vi "Battery_Test_System_Main.vi"() -> ()   [LabVIEW 2019]
doc: "Battery Test System - SIMULATION MODE. One While Loop: Event Structure (UI commands, timeout = UI Update Interval) -> state Case Structure (INIT, IDLE/STOPPED/FAULT, CHARGING/DISCHARGING completion, Default safe fallback) -> Sim_Update_Model (simulated sensor source and output interlock) -> Sim_Check_Safety (latched faults) -> bounded log -> XY graphs and indicators. dt is measured with Tick Count and clamped to Max dt. No physical I/O anywhere. All limits are DEMONSTRATION values only."
uses:
  Sim_Settings.ctl
  Test_State_Enum2.ctl
  Sim_State_Enum.ctl
panel:
  out "Status Message":string
  out "Fault Message":string
  out "Fault":bool
  out "Sim DC Load Output":bool
  out "Sim Power Supply Output":bool
  out "Cycle Count":u32
  out "Elapsed Time (s)":dbl
  out "Temperature (degC)":dbl
  out "DC Current (A)":dbl
  out "DC Voltage (V)":dbl
  out "SOC (%)":dbl
  out "Temperature Graph":T1(graph)
  out "DC Current Graph":cluster{"Time (s)":dbl[], "Current (A)":dbl[]}(graph)
  out "DC Voltage Graph":cluster{"Time (s)":dbl[], "Voltage (V)":dbl[]}(graph)
  out "Current State":T2
  in  "Close":bool
  in  "Reset Fault":bool
  in  "Save":bool
  in  "Stop":bool
  in  "Discharge Settings":T3={"Voltage (V)"=11.0, "Current (A)"=5.0, "C-Rate (1/h)"=1.0, "Duration (min)"=10.0}
  in  "Charge Settings":T3={"Voltage (V)"=14.0, "Current (A)"=5.0, "C-Rate (1/h)"=1.0, "Duration (min)"=10.0}
  in  "Start":bool
  in  "Operation Mode":T4
  in  "Simulation Settings (DEMO ONLY)":T5={"UI Update Interval (ms)"=200, "Max dt (s)"=1.0, "Initial SOC (%)"=50.0, "Rest Voltage (V)"=12.0, "Ambient Temperature (degC)"=25.0, "Voltage Time Constant (s)"=5.0, "Current Time Constant (s)"=1.0, "Thermal Time Constant (s)"=120.0, "Heating Coefficient (degC/s per A^2)"=0.002, "SOC Speed Factor"=1.0, "Charge Complete SOC (%)"=100.0, "Discharge Complete SOC (%)"=0.0, "Max Voltage Limit (V)"=15.0, "Max Current Limit (A)"=10.0, "Max Temperature Limit (degC)"=45.0, "Max C-Rate (1/h)"=5.0, "Max Duration (min)"=600.0, "History Length (samples)"=3000, "Inject E-Stop"=FALSE, "Inject Overvoltage"=FALSE, "Inject Overcurrent"=FALSE, "Inject Overtemperature"=FALSE}
  out "DC Load Connected?":bool
  out "Power Supply Connected?":bool
  out "DAQ CONNECTED?":bool
  out "SIMULATION MODE":string
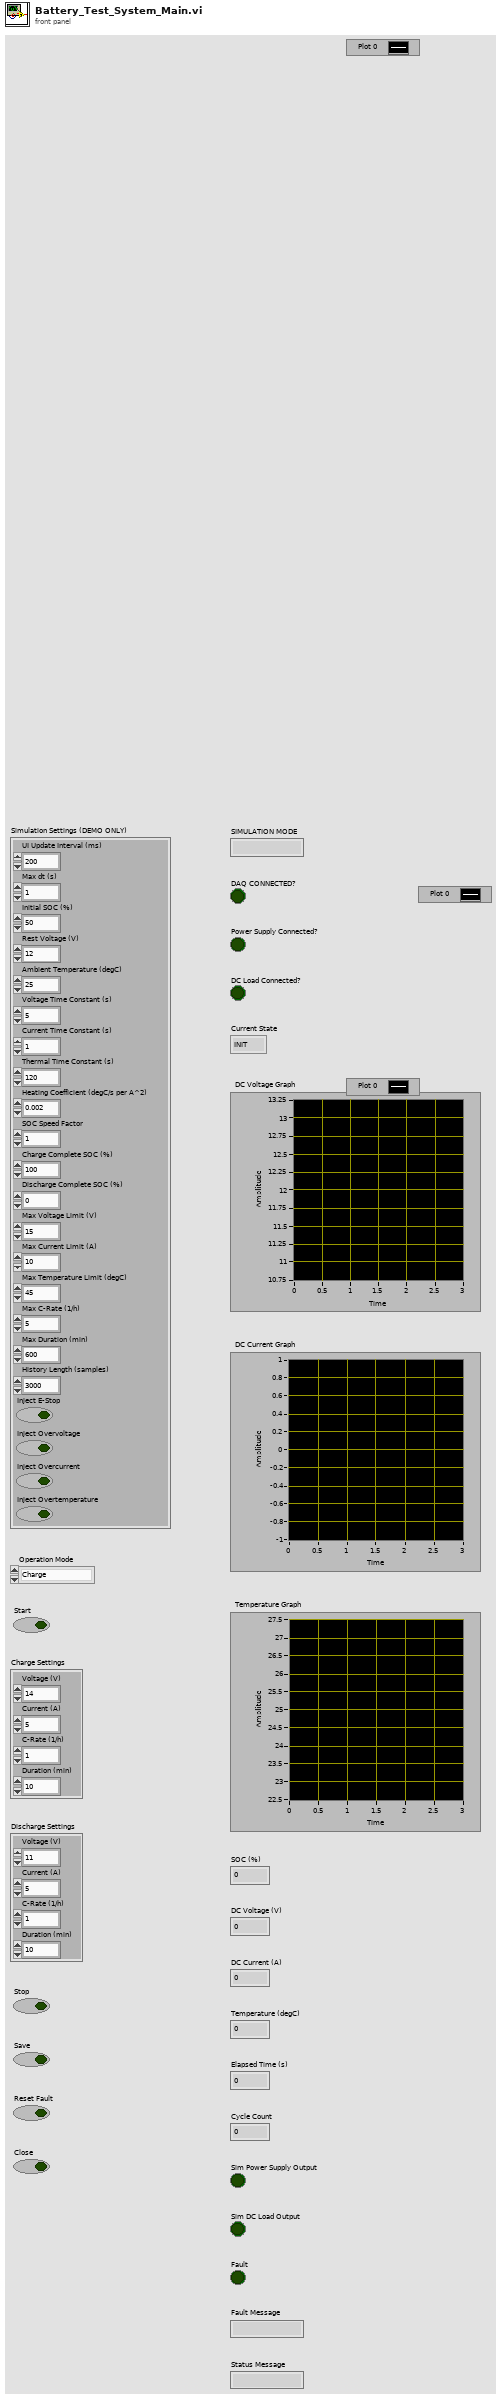
[diagram p1: front panel]
types:
  T1 = cluster{"Time (s)":dbl[], "Temperature (degC)":dbl[]}
  T2 = typedef "Sim_State_Enum.ctl" = enum16{"INIT", "IDLE", "CHARGING", "DISCHARGING", "STOPPED", "FAULT"}
  T3 = cluster{"Voltage (V)":dbl, "Current (A)":dbl, "C-Rate (1/h)":dbl, "Duration (min)":dbl}
  T4 = typedef "Test_State_Enum2.ctl" = enum16{"Charge", "Discharge"}
  T5 = typedef "Sim_Settings.ctl" = cluster{"UI Update Interval (ms)":i32, "Max dt (s)":dbl, "Initial SOC (%)":dbl, "Rest Voltage (V)":dbl, "Ambient Temperature (degC)":dbl, "Voltage Time Constant (s)":dbl, "Current Time Constant (s)":dbl, "Thermal Time Constant (s)":dbl, "Heating Coefficient (degC/s per A^2)":dbl, "SOC Speed Factor":dbl, "Charge Complete SOC (%)":dbl, "Discharge Complete SOC (%)":dbl, "Max Voltage Limit (V)":dbl, "Max Current Limit (A)":dbl, "Max Temperature Limit (degC)":dbl, "Max C-Rate (1/h)":dbl, "Max Duration (min)":dbl, "History Length (samples)":i32, "Inject E-Stop":bool, "Inject Overvoltage":bool, "Inject Overcurrent":bool, "Inject Overtemperature":bool}
  T6 = cluster{"Timestamp":string, "State":enum16{"INIT", "IDLE", "CHARGING", "DISCHARGING", "STOPPED", "FAULT"}, "Data":cluster{"SOC (%)":dbl, "Voltage (V)":dbl, "Current (A)":dbl, "Temperature (degC)":dbl, "Run Time (s)":dbl, "Elapsed (s)":dbl, "Cycle Count":u32, "Active Mode":enum16{"Charge", "Discharge"}, "Setpoint Voltage (V)":dbl, "Setpoint Current (A)":dbl, "Setpoint C-Rate (1/h)":dbl, "Setpoint Duration (min)":dbl, "Sim PS Enable":bool, "Sim Load Enable":bool, "Charge Half Done":bool, "Discharge Half Done":bool, "Fault":bool, "Fault Code":i32, "Fault Message":string, "Fault Time":string, "Status Message":string}}[]
  T7 = cluster{"SOC (%)":dbl, "Voltage (V)":dbl, "Current (A)":dbl, "Temperature (degC)":dbl, "Run Time (s)":dbl, "Elapsed (s)":dbl, "Cycle Count":u32, "Active Mode":enum16{"Charge", "Discharge"}, "Setpoint Voltage (V)":dbl, "Setpoint Current (A)":dbl, "Setpoint C-Rate (1/h)":dbl, "Setpoint Duration (min)":dbl, "Sim PS Enable":bool, "Sim Load Enable":bool, "Charge Half Done":bool, "Discharge Half Done":bool, "Fault":bool, "Fault Code":i32, "Fault Message":string, "Fault Time":string, "Status Message":string}
  T8 = enum16{"INIT", "IDLE", "CHARGING", "DISCHARGING", "STOPPED", "FAULT"}
  T9 = cluster{"Timestamp":string, "State":enum16{"INIT", "IDLE", "CHARGING", "DISCHARGING", "STOPPED", "FAULT"}, "Data":cluster{"SOC (%)":dbl, "Voltage (V)":dbl, "Current (A)":dbl, "Temperature (degC)":dbl, "Run Time (s)":dbl, "Elapsed (s)":dbl, "Cycle Count":u32, "Active Mode":enum16{"Charge", "Discharge"}, "Setpoint Voltage (V)":dbl, "Setpoint Current (A)":dbl, "Setpoint C-Rate (1/h)":dbl, "Setpoint Duration (min)":dbl, "Sim PS Enable":bool, "Sim Load Enable":bool, "Charge Half Done":bool, "Discharge Half Done":bool, "Fault":bool, "Fault Code":i32, "Fault Message":string, "Fault Time":string, "Status Message":string}}
  T10 = typedef "Sim_Data.ctl" = cluster{"SOC (%)":dbl, "Voltage (V)":dbl, "Current (A)":dbl, "Temperature (degC)":dbl, "Run Time (s)":dbl, "Elapsed (s)":dbl, "Cycle Count":u32, "Active Mode":T4, "Setpoint Voltage (V)":dbl, "Setpoint Current (A)":dbl, "Setpoint C-Rate (1/h)":dbl, "Setpoint Duration (min)":dbl, "Sim PS Enable":bool, "Sim Load Enable":bool, "Charge Half Done":bool, "Discharge Half Done":bool, "Fault":bool, "Fault Code":i32, "Fault Message":string, "Fault Time":string, "Status Message":string}
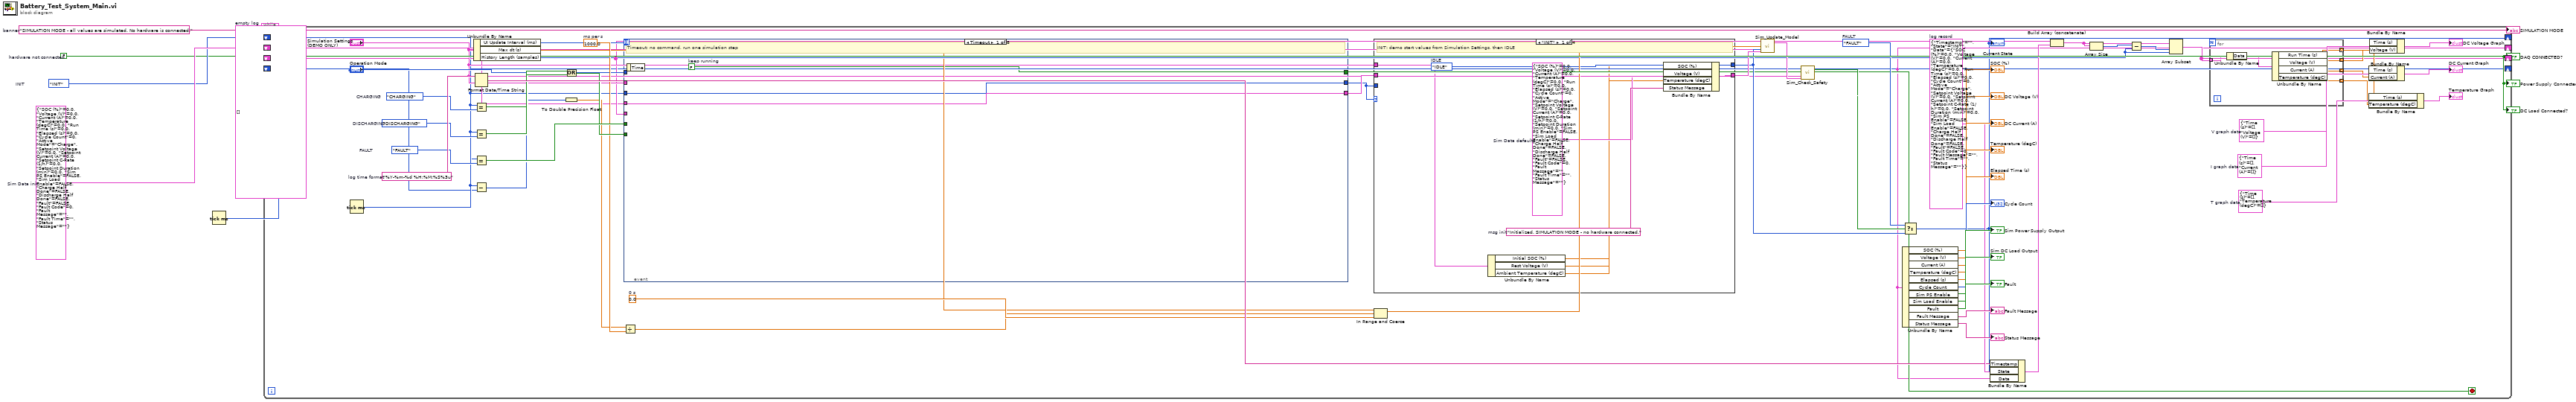
[diagram p0: block diagram]
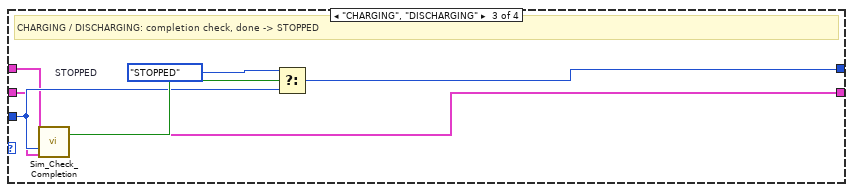
[diagram p3: hidden frame]
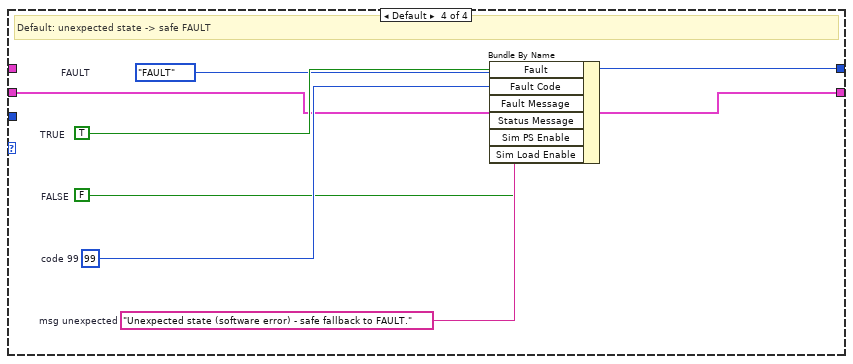
[diagram p4: hidden frame]
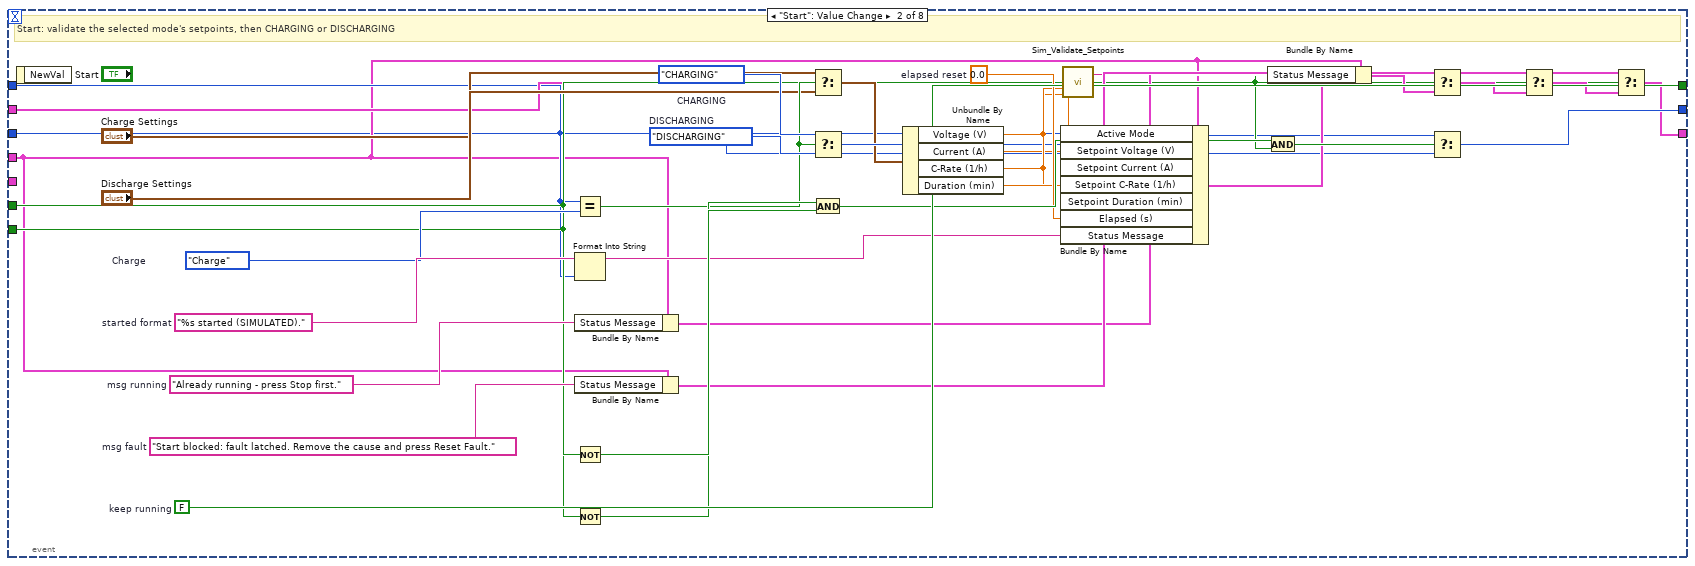
[diagram p5: hidden frame]
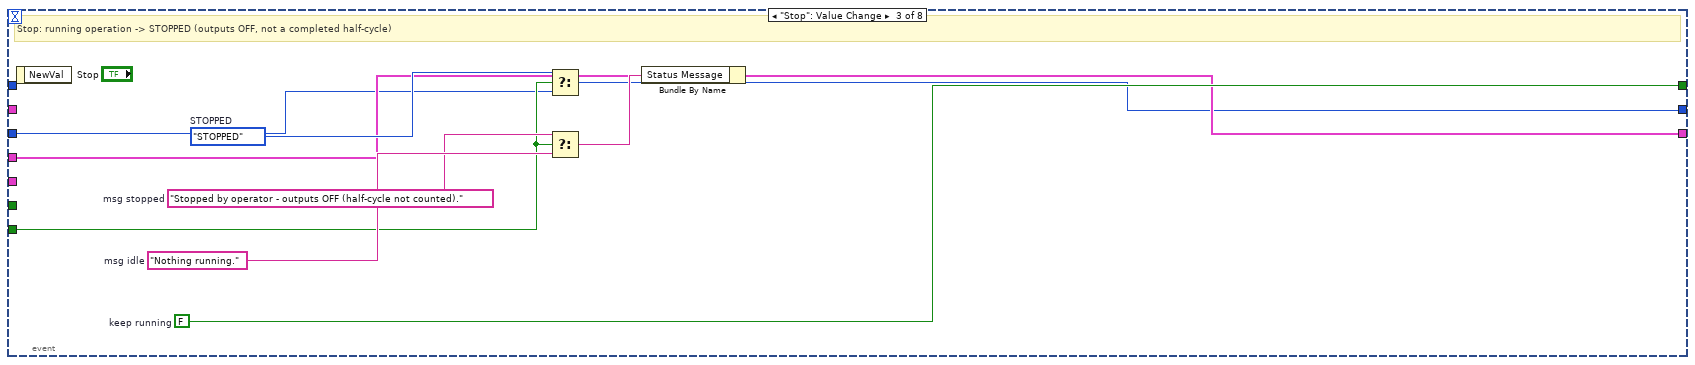
[diagram p6: hidden frame]
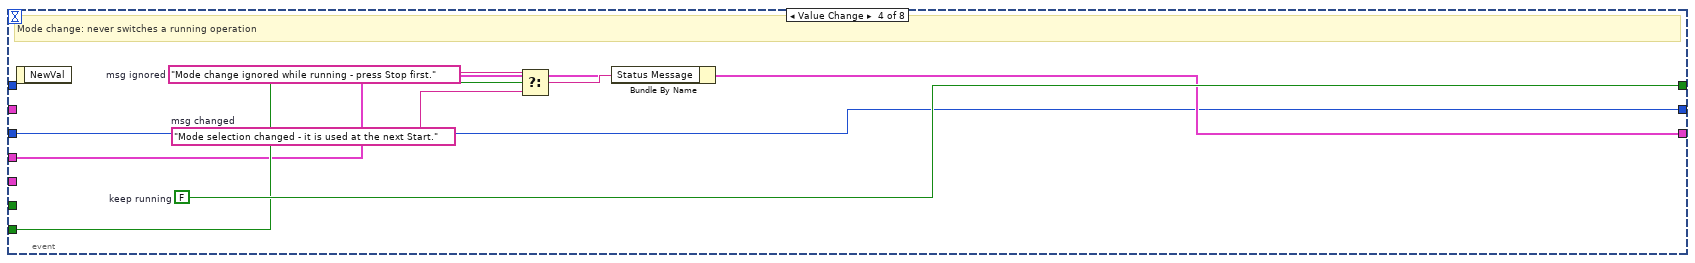
[diagram p7: hidden frame]
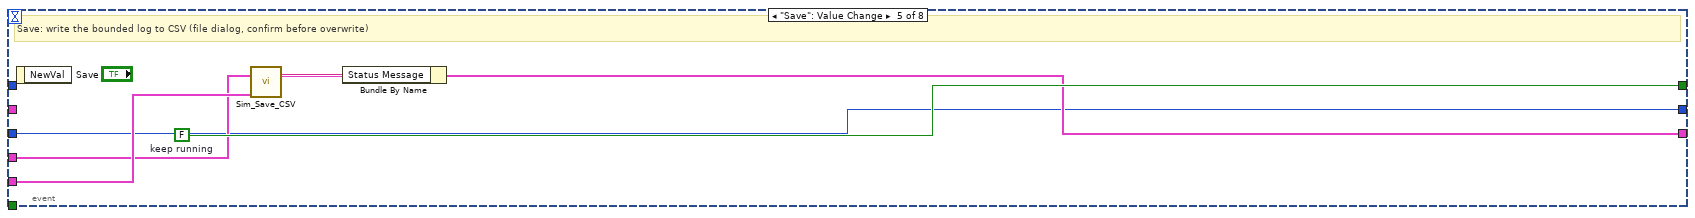
[diagram p8: hidden frame]
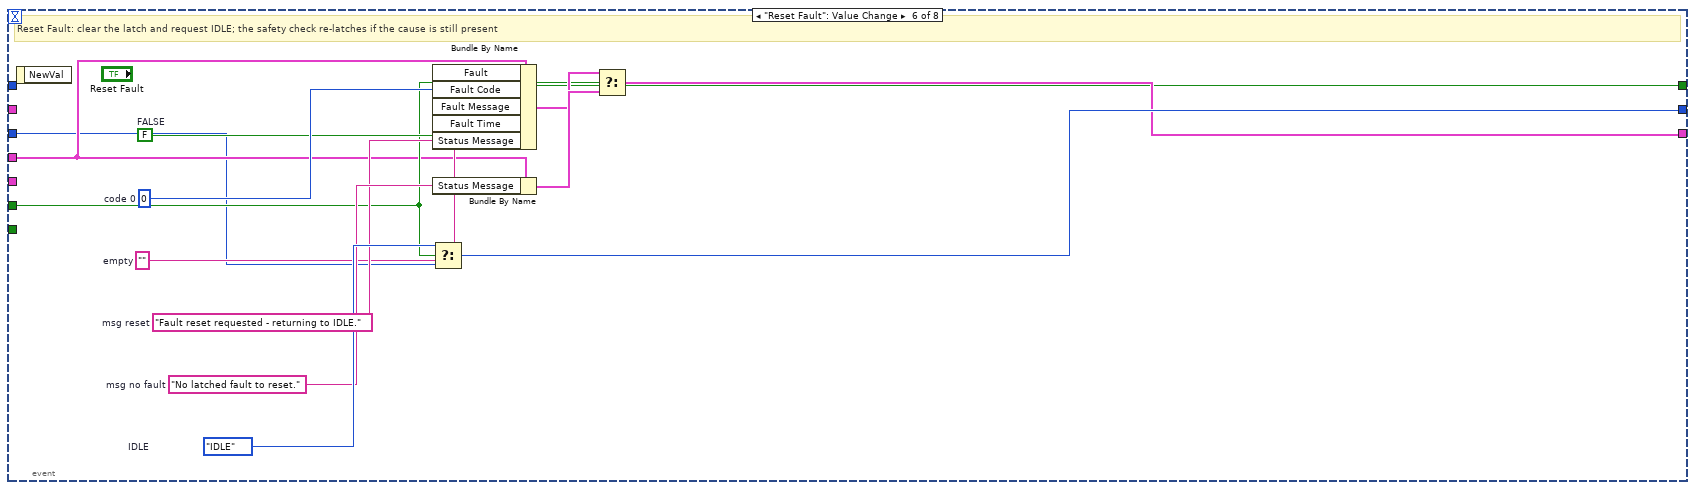
[diagram p9: hidden frame]
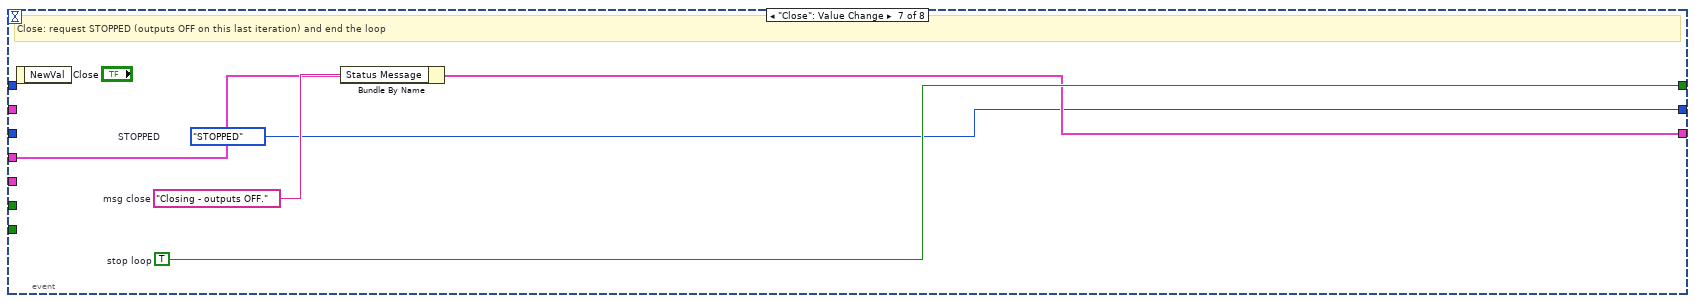
[diagram p10: hidden frame]
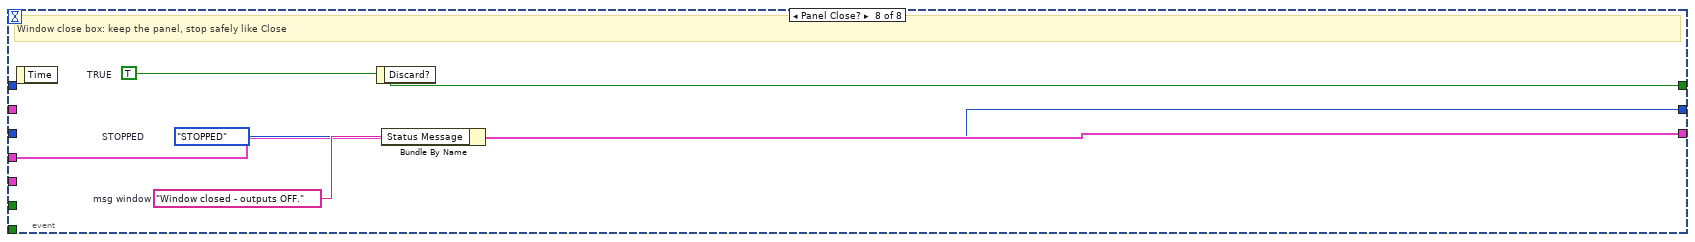
[diagram p11: hidden frame]
diagram:
  w6 = T6 []  # empty log
  w4 = T7 {"SOC (%)"=0.0, "Voltage (V)"=0.0, "Current (A)"=0.0, "Temperature (degC)"=0.0, "Run Time (s)"=0.0, "Elapsed (s)"=0.0, "Cycle Count"=0, "Active Mode"=enum."Charge", "Setpoint Voltage (V)"=0.0, "Setpoint Current (A)"=0.0, "Setpoint C-Rate (1/h)"=0.0, "Setpoint Duration (min)"=0.0, "Sim PS Enable"=FALSE, "Sim Load Enable"=FALSE, "Charge Half Done"=FALSE, "Discharge Half Done"=FALSE, "Fault"=FALSE, "Fault Code"=0, "Fault Message"="", "Fault Time"="", "Status Message"=""}  # Sim Data init
  w3 = T8."INIT"  # INIT
  w2 = FALSE  # hardware not connected
  w1 = "SIMULATION MODE - all values are simulated. No hardware is connected."  # banner
  n1 = Tick Count (ms)() -> (millisecond timer value=w5:u32)
  n2 = while {
    shift-right: [w8] -> _
    shift-left: w3 -> [w7]
    shift-right: [w10] -> _
    shift-left: w4 -> [w9]
    shift-right: [w14] -> _
    shift-left: w6 -> [w13]
    shift-right: [w12] -> _
    shift-left: w5 -> [w11]
    stop <- w35 stop-if-true
    w56 = T1 {"Time (s)"=[], "Temperature (degC)"=[]}  # T graph data
    w54 = cluster{"Time (s)":dbl[], "Current (A)":dbl[]} {"Time (s)"=[], "Current (A)"=[]}  # I graph data
    w52 = cluster{"Time (s)":dbl[], "Voltage (V)":dbl[]} {"Time (s)"=[], "Voltage (V)"=[]}  # V graph data
    w43 = T9 {"Timestamp"="", "State"=enum."INIT", "Data"={"SOC (%)"=0.0, "Voltage (V)"=0.0, "Current (A)"=0.0, "Temperature (degC)"=0.0, "Run Time (s)"=0.0, "Elapsed (s)"=0.0, "Cycle Count"=0, "Active Mode"=enum."Charge", "Setpoint Voltage (V)"=0.0, "Setpoint Current (A)"=0.0, "Setpoint C-Rate (1/h)"=0.0, "Setpoint Duration (min)"=0.0, "Sim PS Enable"=FALSE, "Sim Load Enable"=FALSE, "Charge Half Done"=FALSE, "Discharge Half Done"=FALSE, "Fault"=FALSE, "Fault Code"=0, "Fault Message"="", "Fault Time"="", "Status Message"=""}}  # log record
    w41 = "%Y-%m-%d %H:%M:%S%3u"  # log time format
    w40 = T8."FAULT"  # FAULT
    w28 = T8."FAULT"  # FAULT
    w27 = T8."DISCHARGING"  # DISCHARGING
    w26 = T8."CHARGING"  # CHARGING
    w24 = 0.0  # 0 s
    w22 = 1000.0  # ms per s
    n3 = Tick Count (ms)() -> (millisecond timer value=w12:u32)
    n4 = Unbundle By Name("Simulation Settings (DEMO ONLY)") -> ("UI Update Interval (ms)"=w17:i32, "Max dt (s)"=w18:dbl, "History Length (samples)"=w19:i32)
    n5 = Format Date/Time String(time format string (%c)=w41) -> (date/time string=w42:string)  [unwired: 1 in, 1 out]
    n6 = Equal?(x=w7, y=w26) -> (x = y?=w29:bool)
    n7 = Equal?(x=w7, y=w27) -> (x = y?=w30:bool)
    n8 = Equal?(x=w7, y=w28) -> (x = y?=w32:bool)
    n9 = Subtract(x=w12, y=w11) -> (x-y=w20:u32)
    n10 = Or(x=w29, y=w30) -> (x .or. y?=w31:bool)
    n11 = To Double Precision Float(number=w20) -> (double precision float=w21:dbl)
    n12 = event shown="[0] Timeout" {
      selector: _ -> [_ _ _ _ _ _ _ _]
      dyn-events: _ -> [_ _ _ _ _ _ _ _]
      timeout: w17 -> [_ _ _ _ _ _ _ _]
      tunnel: "Operation Mode" -> [_ w104 _ _ _ _ _ _]
      tunnel: "Simulation Settings (DEMO ONLY)" -> [_ w105 _ _ _ _ _ _]
      tunnel: [w101 w139 w149 w157 w163 w167 w181 w183] -> w35
      tunnel: w7 -> [w99 w102 w140 w150 w158 w164 _ _]
      tunnel: w9 -> [w100 w103 w141 w151 w159 w165 w177 w182]
      tunnel: w13 -> [_ _ _ _ w160 _ _ _]
      tunnel: w32 -> [_ w107 _ _ _ w166 _ _]
      tunnel: [w99 w138 w144 w150 w158 w176 w178 w184] -> w33
      tunnel: [w100 w133 w148 w156 w162 w174 w180 w186] -> w34
      tunnel: w31 -> [_ w106 w142 w152 _ _ _ _]
      event Timeout {
        w101 = FALSE  # keep running
        # "Timeout: no command, run one simulation step"
        n13 = event-data() -> ()  [unwired: 1 in, 1 out]
      }
      event "Start": Value Change {
        w139 = FALSE  # keep running
        w129 = "Start blocked: fault latched. Remove the cause and press Reset Fault."  # msg fault
        w127 = "Already running - press Stop first."  # msg running
        w124 = 0.0  # elapsed reset
        w122 = "%s started (SIMULATED)."  # started format
        w114 = T8."DISCHARGING"  # DISCHARGING
        w113 = T8."CHARGING"  # CHARGING
        w110 = enum16{"Charge", "Discharge"}."Charge"  # Charge
        # "Start: validate the selected mode's setpoints, then CHARGING or DISCHARGING"
        n14 = event-data() -> ()  [unwired: 1 in, 1 out]
        n15 = Equal?(x=w104, y=w110) -> (x = y?=w111:bool)
        n16 = Format Into String(format string=w122, w104) -> (resulting string=w123:string)  [unwired: 2 in, 1 out]
        n17 = Bundle By Name(cluster=w103, "Status Message"=w127) -> (w128:T10)
        n18 = Bundle By Name(cluster=w103, "Status Message"=w129) -> (w130:T10)
        n19 = Not(x=w107) -> (.not. x?=w135:bool)
        n20 = Not(x=w106) -> (.not. x?=w134:bool)
        n21 = Select(t="Charge Settings", s=w111, f="Discharge Settings") -> (s? t:f=w112:T3)
        n22 = Select(t=w113, s=w111, f=w114) -> (s? t:f=w115:T8)
        n23 = And(x=w134, y=w135) -> (x .and. y?=w136:bool)
        n24 = Unbundle By Name(w112) -> ("Voltage (V)"=w116:dbl, "Current (A)"=w117:dbl, "C-Rate (1/h)"=w118:dbl, "Duration (min)"=w119:dbl)
        n25 = Bundle By Name(cluster=w103, "Active Mode"=w104, "Setpoint Voltage (V)"=w116, "Setpoint Current (A)"=w117, "Setpoint C-Rate (1/h)"=w118, "Setpoint Duration (min)"=w119, "Elapsed (s)"=w124, "Status Message"=w123) -> (w125:T10)
        n26 = call "Sim_Validate_Setpoints.vi"("Settings"=w105, "Duration (min)"=w119, "C-Rate (1/h)"=w118, "Current (A)"=w117, "Voltage (V)"=w116) -> ("Message"=w121:string, "Valid?"=w120:bool)  [unwired: 9 in]
        n27 = Bundle By Name(cluster=w103, "Status Message"=w121) -> (w126:T10)
        n28 = And(x=w136, y=w120) -> (x .and. y?=w137:bool)
        n29 = Select(t=w125, s=w120, f=w126) -> (s? t:f=w131:T10)
        n30 = Select(t=w115, s=w137, f=w102) -> (s? t:f=w138:T8)
        n31 = Select(t=w130, s=w107, f=w131) -> (s? t:f=w132:T10)
        n32 = Select(t=w128, s=w106, f=w132) -> (s? t:f=w133:T10)
      }
      event "Stop": Value Change {
        w149 = FALSE  # keep running
        w146 = "Nothing running."  # msg idle
        w145 = "Stopped by operator - outputs OFF (half-cycle not counted)."  # msg stopped
        w143 = T8."STOPPED"  # STOPPED
        # "Stop: running operation -> STOPPED (outputs OFF, not a completed half-cycle)"
        n33 = event-data() -> ()  [unwired: 1 in, 1 out]
        n34 = Select(t=w143, s=w142, f=w140) -> (s? t:f=w144:T8)
        n35 = Select(t=w145, s=w142, f=w146) -> (s? t:f=w147:string)
        n36 = Bundle By Name(cluster=w141, "Status Message"=w147) -> (w148:T10)
      }
      event Value Change {
        w157 = FALSE  # keep running
        w154 = "Mode selection changed - it is used at the next Start."  # msg changed
        w153 = "Mode change ignored while running - press Stop first."  # msg ignored
        # "Mode change: never switches a running operation"
        n37 = event-data() -> ()  [unwired: 1 in, 1 out]
        n38 = Select(t=w153, s=w152, f=w154) -> (s? t:f=w155:string)
        n39 = Bundle By Name(cluster=w151, "Status Message"=w155) -> (w156:T10)
      }
      event "Save": Value Change {
        w163 = FALSE  # keep running
        # "Save: write the bounded log to CSV (file dialog, confirm before overwrite)"
        n40 = event-data() -> ()  [unwired: 1 in, 1 out]
        n41 = call "Sim_Save_CSV.vi"("Log Records"=w160) -> ("Status Message"=w161:string)  [unwired: 13 in, 1 out]
        n42 = Bundle By Name(cluster=w159, "Status Message"=w161) -> (w162:T10)
      }
      event "Reset Fault": Value Change {
        w175 = T8."IDLE"  # IDLE
        w171 = "No latched fault to reset."  # msg no fault
        w170 = "Fault reset requested - returning to IDLE."  # msg reset
        w169 = ""  # empty
        w168 = 0  # code 0
        w167 = FALSE  # FALSE
        # "Reset Fault: clear the latch and request IDLE; the safety check re-latches if the cause is still present"
        n43 = event-data() -> ()  [unwired: 1 in, 1 out]
        n44 = Bundle By Name(cluster=w165, "Fault"=w167, "Fault Code"=w168, "Fault Message"=w169, "Fault Time"=w169, "Status Message"=w170) -> (w172:T10)
        n45 = Bundle By Name(cluster=w165, "Status Message"=w171) -> (w173:T10)
        n46 = Select(t=w175, s=w166, f=w164) -> (s? t:f=w176:T8)
        n47 = Select(t=w172, s=w166, f=w173) -> (s? t:f=w174:T10)
      }
      event "Close": Value Change {
        w181 = TRUE  # stop loop
        w179 = "Closing - outputs OFF."  # msg close
        w178 = T8."STOPPED"  # STOPPED
        # "Close: request STOPPED (outputs OFF on this last iteration) and end the loop"
        n48 = event-data() -> ()  [unwired: 1 in, 1 out]
        n49 = Bundle By Name(cluster=w177, "Status Message"=w179) -> (w180:T10)
      }
      event Panel Close? {
        w185 = "Window closed - outputs OFF."  # msg window
        w184 = T8."STOPPED"  # STOPPED
        w183 = TRUE  # TRUE
        # "Window close box: keep the panel, stop safely like Close"
        n50 = event-data() -> ()  [unwired: 1 in, 1 out]
        n51 = event-data("Discard?"=w183) -> ()  [unwired: 1 in, 1 out]
        n52 = Bundle By Name(cluster=w182, "Status Message"=w185) -> (w186:T10)
      }
    }
    n53 = Divide(x=w21, y=w22) -> (x/y=w23:dbl)
    n54 = case shown="\"INIT\"" w33 {
      tunnel: "Simulation Settings (DEMO ONLY)" -> [w75 _ w86 _]
      tunnel: [w82 w84 w91 w93] -> w36
      tunnel: w34 -> [_ w83 w85 w92]
      tunnel: w33 -> [_ w84 w87 _]
      tunnel: [w81 w83 w88 w98] -> w37
      frame "INIT" {
        w82 = T8."IDLE"  # IDLE
        w80 = "Initialized. SIMULATION MODE - no hardware connected."  # msg init
        w79 = T7 {"SOC (%)"=0.0, "Voltage (V)"=0.0, "Current (A)"=0.0, "Temperature (degC)"=0.0, "Run Time (s)"=0.0, "Elapsed (s)"=0.0, "Cycle Count"=0, "Active Mode"=enum."Charge", "Setpoint Voltage (V)"=0.0, "Setpoint Current (A)"=0.0, "Setpoint C-Rate (1/h)"=0.0, "Setpoint Duration (min)"=0.0, "Sim PS Enable"=FALSE, "Sim Load Enable"=FALSE, "Charge Half Done"=FALSE, "Discharge Half Done"=FALSE, "Fault"=FALSE, "Fault Code"=0, "Fault Message"="", "Fault Time"="", "Status Message"=""}  # Sim Data defaults
        # "INIT: demo start values from Simulation Settings, then IDLE"
        n55 = Unbundle By Name(w75) -> ("Initial SOC (%)"=w76:dbl, "Rest Voltage (V)"=w77:dbl, "Ambient Temperature (degC)"=w78:dbl)
        n56 = Bundle By Name(cluster=w79, "SOC (%)"=w76, "Voltage (V)"=w77, "Temperature (degC)"=w78, "Status Message"=w80) -> (w81:T7)
      }
      frame "IDLE", "STOPPED", "FAULT" {
        # "IDLE / STOPPED / FAULT: hold; the model forces both outputs OFF"
      }
      frame "CHARGING", "DISCHARGING" {
        w90 = T8."STOPPED"  # STOPPED
        # "CHARGING / DISCHARGING: completion check, done -> STOPPED"
        n57 = call "Sim_Check_Completion.vi"("State"=w87, "Settings"=w86, "Sim Data in"=w85) -> ("Done?"=w89:bool, "Sim Data out"=w88:T10)  [unwired: 11 in]
        n58 = Select(t=w90, s=w89, f=w87) -> (s? t:f=w91:T8)
      }
      frame Default {
        w97 = "Unexpected state (software error) - safe fallback to FAULT."  # msg unexpected
        w96 = 99  # code 99
        w95 = FALSE  # FALSE
        w94 = TRUE  # TRUE
        w93 = T8."FAULT"  # FAULT
        # "Default: unexpected state -> safe FAULT"
        n59 = Bundle By Name(cluster=w92, "Fault"=w94, "Fault Code"=w96, "Fault Message"=w97, "Status Message"=w97, "Sim PS Enable"=w95, "Sim Load Enable"=w95) -> (w98:T10)
      }
    }
    n60 = In Range and Coerce(upper limit=w18, x=w23, lower limit=w24) -> (coerced(x)=w25:dbl)  [unwired: 1 out]
    n61 = call "Sim_Update_Model.vi"("dt (s)"=w25, "State"=w36, "Settings"="Simulation Settings (DEMO ONLY)", "Sim Data in"=w37) -> ("Sim Data out"=w38:T10)  [unwired: 11 in]
    n62 = call "Sim_Check_Safety.vi"("Settings"="Simulation Settings (DEMO ONLY)", "Sim Data in"=w38) -> ("Fault Active?"=w39:bool, "Sim Data out"=w10:T10)  [unwired: 12 in]
    n63 = Unbundle By Name(w10) -> ("SOC (%)"=→"SOC (%)":dbl, "Voltage (V)"=→"DC Voltage (V)":dbl, "Current (A)"=→"DC Current (A)":dbl, "Temperature (degC)"=→"Temperature (degC)":dbl, "Elapsed (s)"=→"Elapsed Time (s)":dbl, "Cycle Count"=→"Cycle Count":u32, "Sim PS Enable"=→"Sim Power Supply Output":bool, "Sim Load Enable"=→"Sim DC Load Output":bool, "Fault"=→"Fault":bool, "Fault Message"=→"Fault Message":string, "Status Message"=→"Status Message":string)
    n64 = Select(t=w40, s=w39, f=w36) -> (s? t:f=w8:T8)
    "Current State" <- w8
    n65 = Bundle By Name(cluster=w43, "Timestamp"=w42, "State"=w8, "Data"=w10) -> (w44:T9)
    n66 = Build Array (concatenate)(w13, w44) -> (w45:T6)
    n67 = Array Size(array=w45) -> (size(s)=w46:i32)
    n68 = Subtract(x=w46, y=w19) -> (x-y=w47:i32)
    n69 = Array Subset(array=w45, index=w47, length=w19) -> (w14:T6)
    n70 = for {
      tunnel: w14 -> [w69] mode=indexing
      tunnel: [w71] -> w48 mode=indexing
      tunnel: [w72] -> w49 mode=indexing
      tunnel: [w73] -> w50 mode=indexing
      tunnel: [w74] -> w51 mode=indexing
      n71 = Unbundle By Name(w69) -> ("Data"=w70:T7)
      n72 = Unbundle By Name(w70) -> ("Run Time (s)"=w71:dbl, "Voltage (V)"=w72:dbl, "Current (A)"=w73:dbl, "Temperature (degC)"=w74:dbl)
    }
    n73 = Bundle By Name(cluster=w56, "Time (s)"=w48, "Temperature (degC)"=w51) -> (→"Temperature Graph":T1)
    n74 = Bundle By Name(cluster=w54, "Time (s)"=w48, "Current (A)"=w50) -> (→"DC Current Graph":cluster{"Time (s)":dbl[], "Current (A)":dbl[]})
    n75 = Bundle By Name(cluster=w52, "Time (s)"=w48, "Voltage (V)"=w49) -> (→"DC Voltage Graph":cluster{"Time (s)":dbl[], "Voltage (V)":dbl[]})
  }
  "SIMULATION MODE" <- w1
  "DAQ CONNECTED?" <- w2
  "Power Supply Connected?" <- w2
  "DC Load Connected?" <- w2
